vi "macro_FlyWheel_Sim_Execute.vi"() -> ()   [LabVIEW 2019, in "Trajectory_Library.lvlib"]
uses:
  Trajectory_Library.lvlib
  Enum/DCMOTOR_TYPES_ENUM.ctl
  BatterySim_CalculateLoadedBatteryVoltage.vi
panel:
  in  "Motor Dmd (CO)":dbl
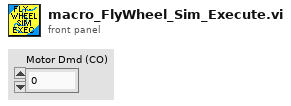
[diagram p1: front panel]
types:
  T1 = typedef "Trajectory_Library.lvlib/DCMOTOR_TYPES_ENUM.ctl" = enum16{"CIM", "AndyMark 9015", "Andy Mark RS 775 125", "Bag", "BaneBots RS 550", "BaneBots RS 775", "Falcon 500", "Mini CIM", "NEO", "NEO 550", "Romi BuiltIn", "Vex 775 Pro", "Snow Blower AM 2235A", "Bosch Seat AM 3493"}
  T2 = typedef "Trajectory_Library.lvlib/LINEAR_SYSTEM_ID_FLYWHEEL_MODEL.ctl" = cluster{"DCMOTOR_TYPES":T1, "Num Motors":i32, "Gearing":dbl, "MOI kgm2":dbl}
  T3 = typedef "Trajectory_Library.lvlib/FLYWHEEL_SIM_SIMULATION_PARAMS.ctl" = cluster{"Vel Meas Std Dev Rad/Sec":dbl}
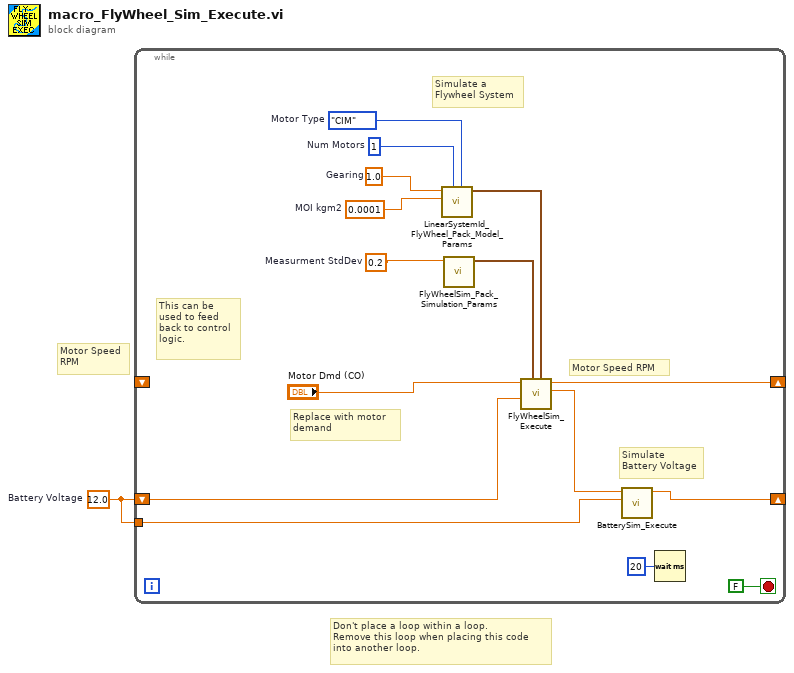
[diagram p0: block diagram]
diagram:
  w1 = 12.0  # Battery Voltage
  # "Don't place a loop within a loop. \nRemove this loop when placing this code\ninto another loop."
  # "Motor Speed\nRPM"
  n1 = while {
    shift-right: [w9] -> _
    shift-left: w1 -> [w6]
    shift-right: [w7] -> _
    shift-left: _ -> [_]
    tunnel: w1 -> [w2]
    stop <- FALSE stop-if-true
    w4 = 0.2  # Measurment StdDev
    w13 = 1.0  # Gearing
    w14 = 0.0001  # MOI kgm2
    w15 = 1  # Num Motors
    w16 = DCMOTOR_TYPES_ENUM."CIM"  # Motor Type
    # "This can be\nused to feed\nback to control\nlogic."
    # "Motor Speed RPM"
    # "Replace with motor \ndemand"
    # "Simulate\nBattery Voltage"
    # "Simulate a \nFlywheel System"
    n2 = call "LinearSystemId_FlyWheel_Pack_Model_Params.vi"("DCMOTOR_TYPES"=w16, "Num Motors"=w15, "MOI kgm2"=w14, "Gearing"=w13) -> ("LinearSystem_ID_FlyWheel_Model"=w5:T2)  [unwired: 7 in]
    n3 = call "FlyWheelSim_Pack_Simulation_Params.vi"("Vel Meas StdDev Rad/Sec"=w4) -> ("FlyWheelSim_Simulation_Params"=w3:T3)  [unwired: 10 in]
    n4 = call "FlyWheelSim_Execute.vi"("FlyWheelSim_Model _Params"=w5, "FlyWheelSim_Simulation_Params"=w3, "Battery Volts"=w6, "Motor Dmd"="Motor Dmd (CO)") -> ("Motor Current"=w10:dbl, "Velocity_RPM"=w7:dbl)  [unwired: 4 in, 2 out]
    n5 = call "BatterySim_Execute.vi"("Nominal Battery Voltage"=w2, "Current"=w10) -> ("Voltage"=w9:dbl)  [unwired: 9 in]
    n6 = Wait (ms)(milliseconds to wait=u32 20) -> ()  [unwired: 1 out]
  }
